vi "GDSProject_SaveProject.vi"(10 "error in (no error)":errorcluster, 11 "Project in":refnum<vi>) -> (2 "error out":errorcluster, 3 "Project out":refnum<vi>)   [LabVIEW 2020]
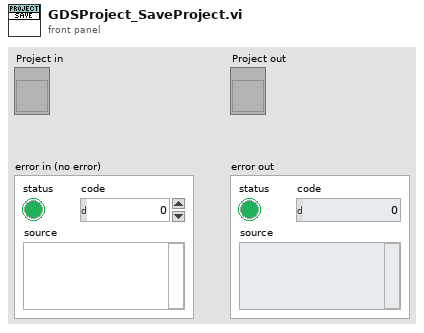
[diagram p1: front panel]
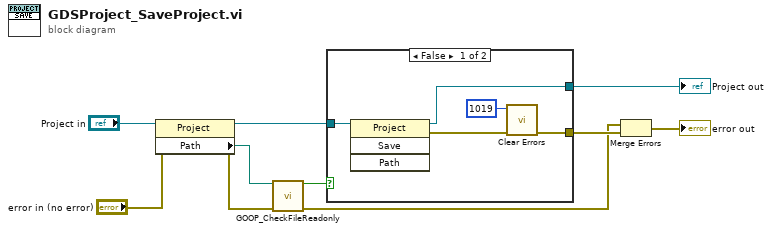
[diagram p0: block diagram]
diagram:
  n1 = property class="Project"(reference="Project in", error in="error in (no error)") -> (reference out=w6:refnum<vi>, error out=w4:errorcluster, "Path"=w2:path)
  n2 = call "GOOP_CheckFileReadonly.vi"("FilePath"=w2, "error in"=w4) -> ("IsReadOnly"=w1:bool, "error out"=w3:errorcluster)  [unwired: 12 in]
  n3 = case shown="False" w1 {
    tunnel: [w15 w16] -> w10
    tunnel: [w12 _] -> w7
    tunnel: w6 -> [w11 w16]
    frame False {
      n4 = invoke class="Project" method="Save"(reference=w11) -> (reference out=w15:refnum<vi>, error out=w13:errorcluster)  [unwired: 3 in, 2 out]
      n5 = call <vilib>:"Clear Errors.vi"("error in (no error)"=w13, "specific error code to clear (0: all)"=1019) -> ("error out"=w12:errorcluster)  [unwired: 4 in, 1 out]
    }
    frame True {
    }
  }
  "Project out" <- w10
  n6 = Merge Errors(w3, w7) -> (→"error out":errorcluster)
